vi "TDMS to TXT Modification.vi"(8 "error in":errorcluster caption="エラー入力（エラーなし）", 11 "Original File name (TDMS)":path) -> (0 "error out":errorcluster caption="エラー出力", 3 "波形グラフ":dbl[](graph))   [LabVIEW 2018]
panel:
  out "Numeric":i32
  out "channel names":string[](array[string])
  out "channel name out":string
  out "path":path
  out "temp txt_path":path
  out "データ":dbl[](array[numeric])
  out "file or folder exists?":bool caption="既存するファイルまたはフォルダ?"
  out "Create File name (TXT)":path
  in  "stop":bool
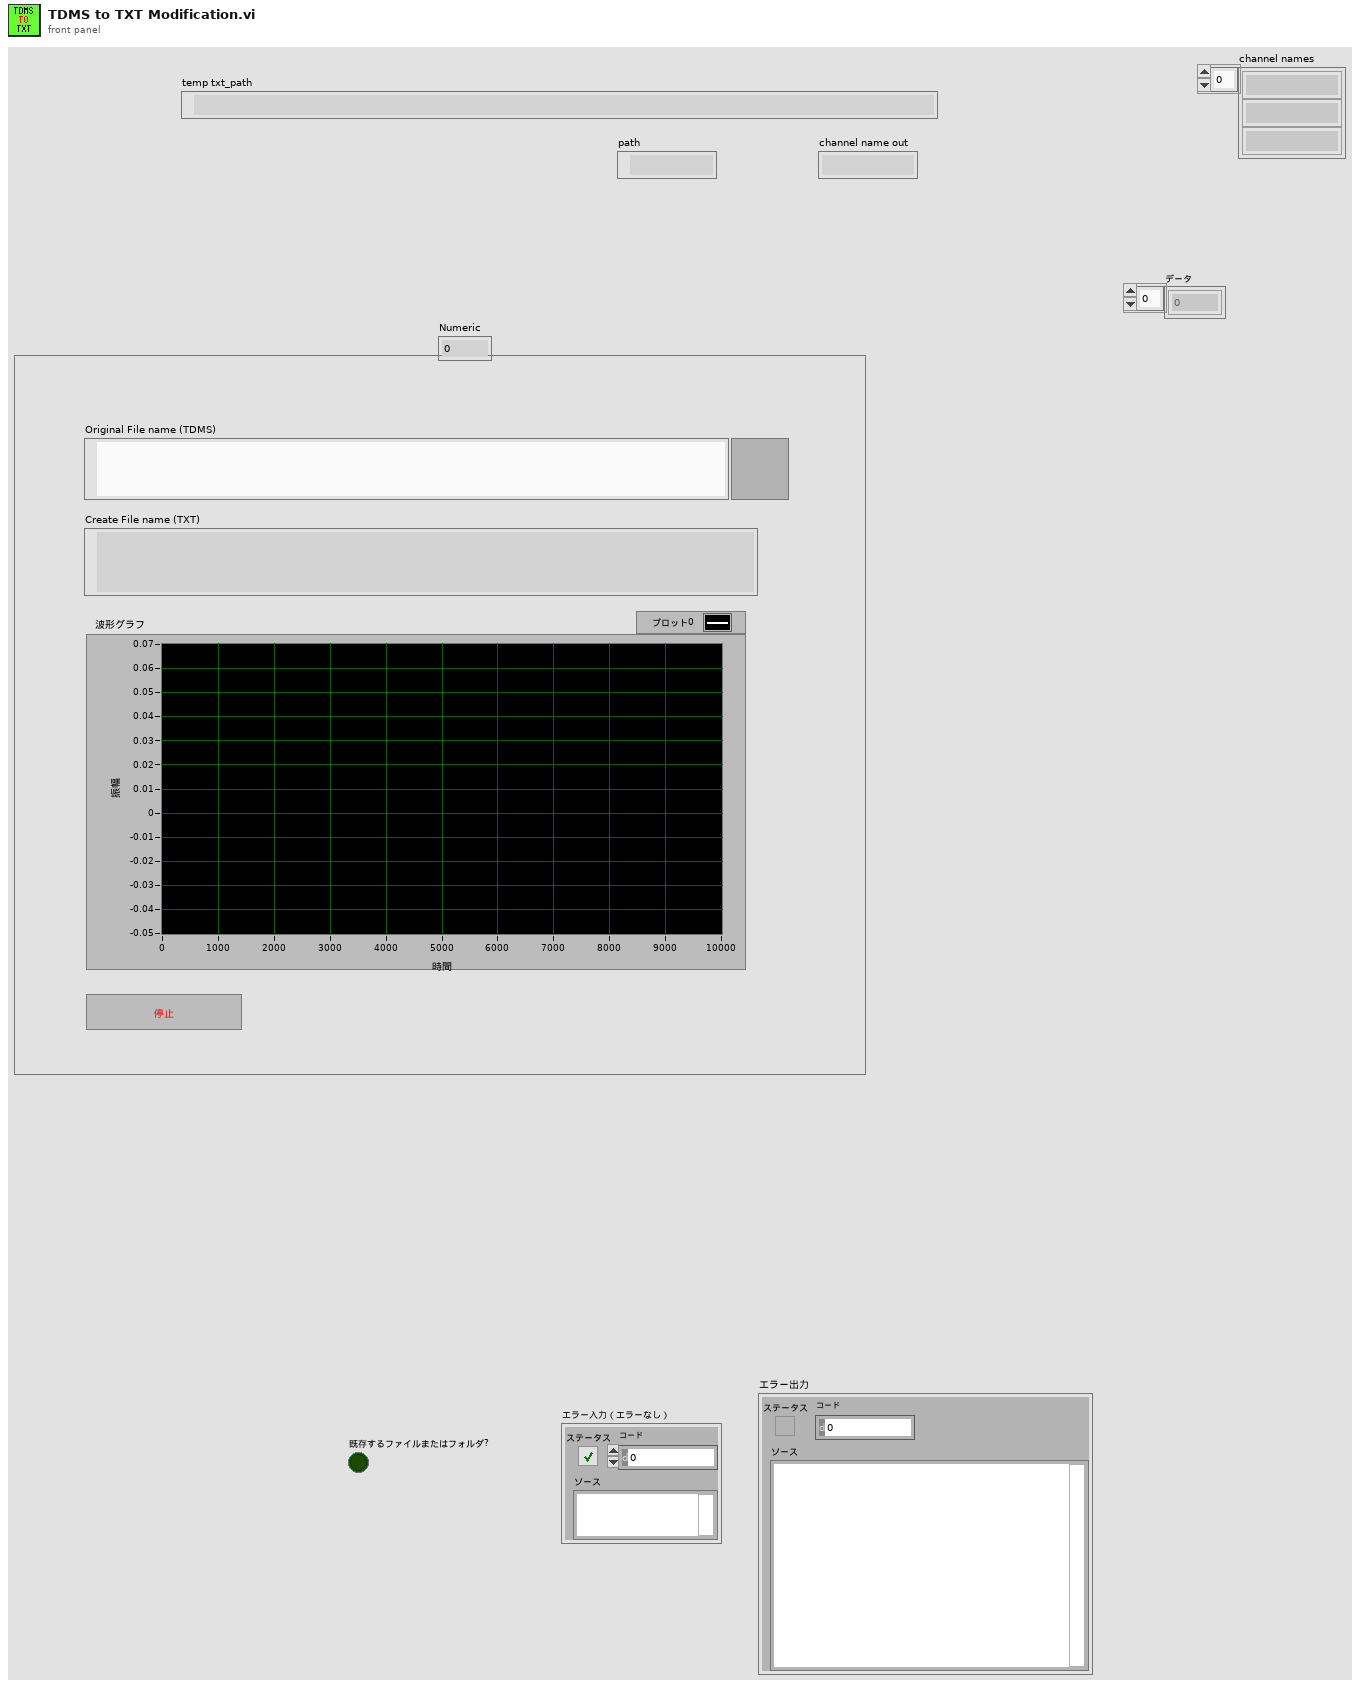
[diagram p1: front panel]
types:
  T1 = enum16{"open", "open or create", "create or replace", "create", "open (read-only)"}
  T2 = enum16{"open", "replace", "create", "open or create", "replace or create", "replace or create with confirmation"}
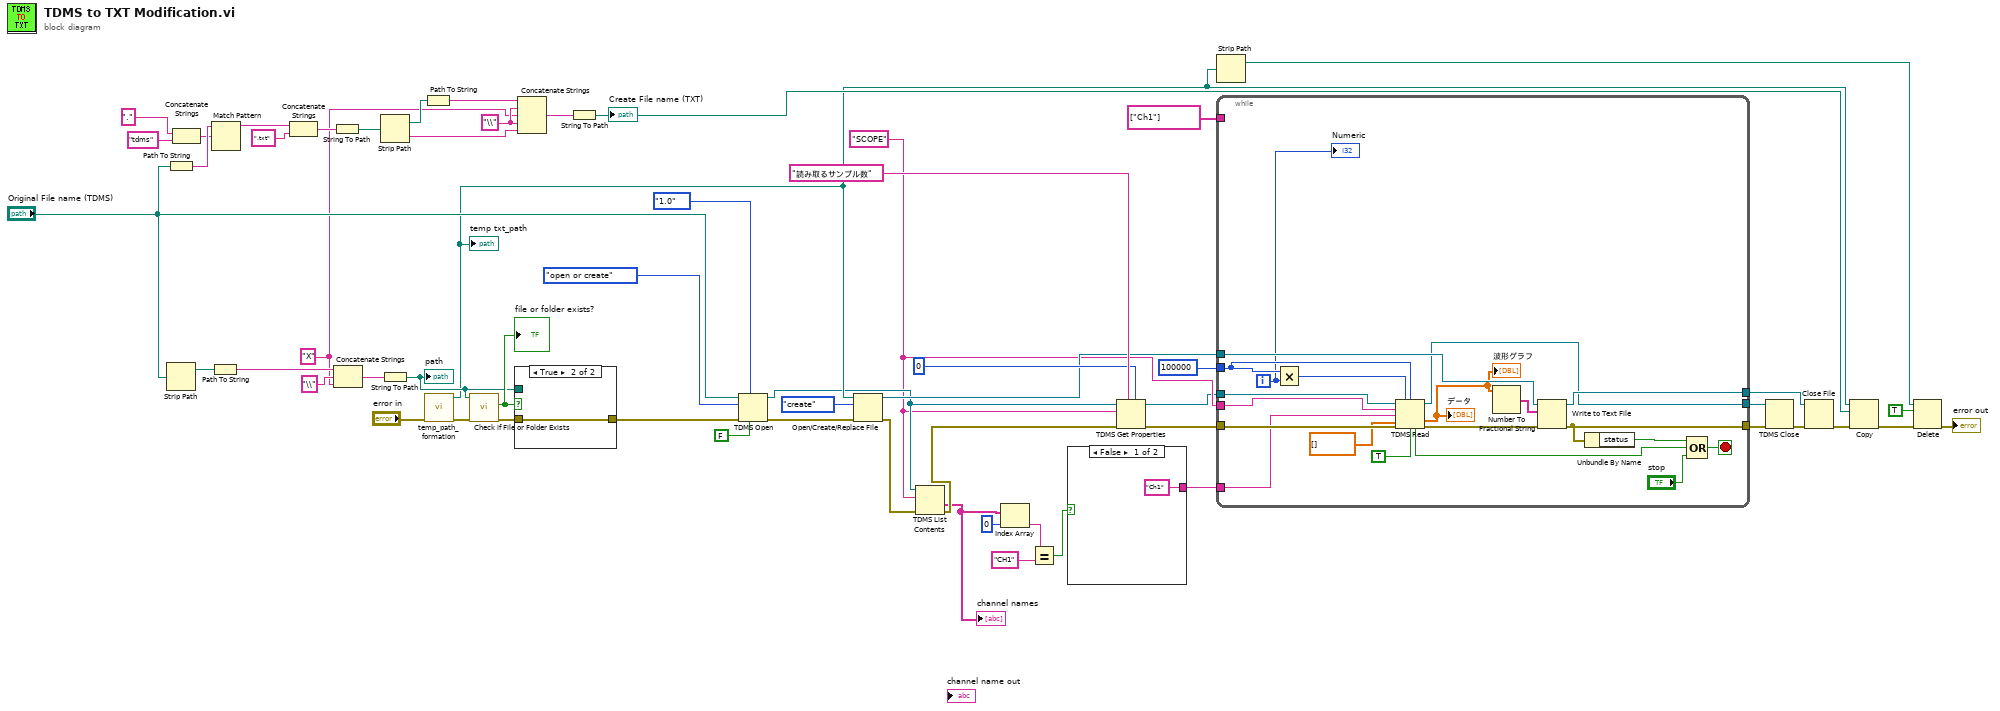
[diagram p0: block diagram]
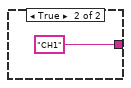
[diagram p2: hidden frame]
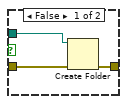
[diagram p3: hidden frame]
diagram:
  w29 = "X" ("Folder Name")
  w38 = "\\" ("文字列")
  w19 = "SCOPE" ("グループ名")
  n1 = Path To String(path="Original File name (TDMS)") -> (string=w50:string)
  n2 = Strip Path(path="Original File name (TDMS)") -> (stripped path=w31:path)  [unwired: 1 out]
  n3 = Concatenate Strings("." ("正規表現"), "tdms" ("File Extention form")) -> (w45:string)
  n4 = Path To String(path=w31) -> (string=w30:string)
  n5 = Match Pattern(string=w50, regular expression=w45) -> (before substring=w49:string)  [unwired: 1 in, 3 out]
  n6 = Concatenate Strings(w49, ".txt" ("文字列")) -> (w48:string)
  n7 = String To Path(string=w48) -> (path=w44:path)
  n8 = Concatenate Strings(w30, "\\" ("文字列"), w29) -> (w34:string)
  n9 = Strip Path(path=w44) -> (stripped path=w43:path, name=w39:string)
  n10 = String To Path(string=w34) -> (path=w35:path)
  "path" <- w35
  n11 = Path To String(path=w43) -> (string=w42:string)
  n12 = call "temp_path_formation.vi"("error in (no error)"="error in") -> ("error out"=w25:errorcluster, "temp txt_path"=w24:path)  [unwired: 8 in, 1 out]
  "temp txt_path" <- w24
  n13 = call <vilib>:"Check if File or Folder Exists.vi"("error in (no error)"=w25, "path"=w35) -> ("error out"=w33:errorcluster, "file or folder exists?"=w37:bool)  [unwired: 7 in, 1 out]
  "file or folder exists?" <- w37
  n14 = case shown="True" w37 {
    tunnel: w35 -> [w61 _]
    tunnel: w33 -> [w60 w62]
    tunnel: [w59 w62] -> w27
    frame False {
      n15 = Create Folder(path (use dialog)=w61, error in=w60) -> (error out=w59:errorcluster)  [unwired: 1 in, 2 out]
    }
    frame True {
    }
  }
  n16 = Concatenate Strings(w42, w38, w29, w38, w39) -> (w41:string)
  n17 = String To Path(string=w41) -> (path=w28:path)
  "Create File name (TXT)" <- w28
  n18 = TDMS Open(6:FALSE ("disable buffering (T)"), 7:enum16{"1.0", "2.0"}."1.0" ("file format version (2.0)"), 8:w27, 10:T1."open or create" ("operation"), 11:"Original File name (TDMS)") -> (0:w51:errorcluster, 3:w20:refnum<k34>)  [unwired: 2 in]
  n19 = Open/Create/Replace File(file path (use dialog)=w24, error in=w51, operation (0:open)=T2."create" ("操作（0:開く）")) -> (refnum out=w56:refnum<file>, error out=w22:errorcluster)  [unwired: 3 in, 1 out]
  n20 = TDMS List Contents(4:w22, 6:w19, 7:w20) -> (0:w21:errorcluster, 1:w6:string[])  [unwired: 2 out]
  "channel names" <- w6
  n21 = Index Array(array=w6, index=0) -> (element=w3:string)
  n22 = Equal?(x=w3, y="CH1") -> (x = y?=w2:bool)
  n23 = case shown="False" w2 {
    tunnel: ["Ch1" ("channel name(s) in") "CH1" ("channel name(s) in")] -> w4
    frame False {
    }
    frame True {
    }
  }
  n24 = TDMS Get Properties(5:u32 0 ("Max Points Per Fetch"), 7:"読み取るサンプル数", 8:w21, 10:w19, 11:w20) -> (0:w15:errorcluster, 3:w16:refnum<k34>)  [unwired: 1 in, 4 out]
  n25 = Strip Path(path=w24) -> (stripped path=w9:path)  [unwired: 1 out]
  n26 = while {
    tunnel: w15 -> [w84]
    tunnel: [w75] -> w18
    tunnel: w16 -> [w83]
    tunnel: [w71] -> w17
    tunnel: u32 100000 ("Max Points Per Fetch") -> [w82]
    tunnel: w56 -> [w74]
    tunnel: [w73] -> w14
    tunnel: string[] ["Ch1"] ("付加配列") -> [_]
    tunnel: w19 -> [w67]
    tunnel: w4 -> [w65]
    i -> [w66]
    stop <- w78 stop-if-true
    n27 = Multiply(x=w82, y=w66) -> (x*y=w81:u32)
    n28 = TDMS Read(0:w83, 1:w81, 2:w82, 5:w67, 7:w65, 11:w84, 12:dbl[] [], 13:TRUE ("ファイル順にチャンネルを返す?（F）")) -> (4:w71:refnum<k34>, 10:w69:dbl[], 14:w70:bool, 15:w76:errorcluster)  [unwired: 2 out]
    "波形グラフ" <- w69
    "データ" <- w69
    n29 = Number To Fractional String(number=w69) -> (F-format string=w72:string[])  [unwired: 3 in]
    n30 = Write to Text File(file (use dialog)=w74, text=w72, error in=w76) -> (refnum out=w73:refnum<file>, error out=w75:errorcluster)  [unwired: 1 in, 1 out]
    n31 = Unbundle By Name(w75) -> ("status"=w80:bool)
    n32 = Compound Arithmetic op=OR(w80, w70, "stop") -> (w78:bool)
    "Numeric" <- w66
  }
  n33 = TDMS Close(8:w18, 11:w17) -> (0:w13:errorcluster)  [unwired: 1 out]
  n34 = Close File(refnum=w14, error in=w13) -> (error out=w10:errorcluster)  [unwired: 1 out]
  n35 = Copy(8:w10, 10:w28, 11:w24) -> (0:w7:errorcluster)  [unwired: 2 in, 2 out]
  n36 = Delete(path (use dialog)=w9, entire hierarchy (F)=TRUE, error in=w7) -> (error out=→"error out":errorcluster)  [unwired: 2 in, 2 out]
